vi "Process Data.vi"(7 "Buffer Length":i32, 8 "error in (no error)":errorcluster, 9 "Data":dbl[](array[numeric])=[nan, nan], 10 "XY Plot":refnum<vi>, 11 "Data Rate":i32 caption="ms") -> (0 "error out":errorcluster)   [LabVIEW 2025, in "H1 Plotter.lvlib" / "H1 Velocity.lvclass"]
uses:
  H1 Velocity.lvclass
  H1 Velocity.lvclass/H1 Velocity.ctl
  Users/Public/Documents/Sandia National Labs/TSS Plugin/Tests/XY Plotter.lvlibp/XY  Plotter/XY Plotter.lvclass
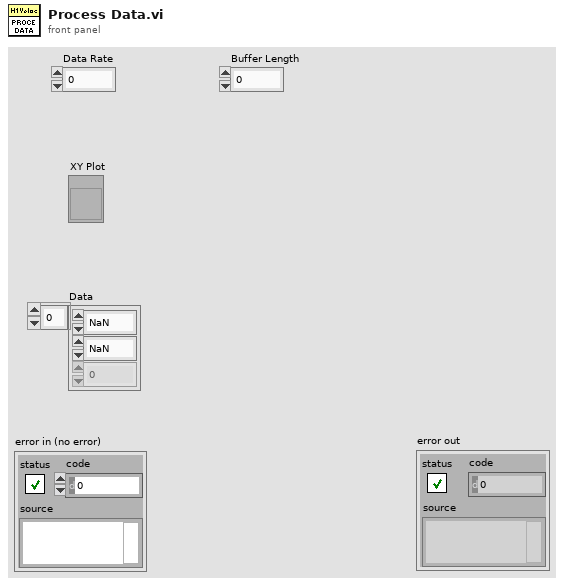
[diagram p1: front panel]
types:
  T1 = cluster{"Active Plot":u32, "XY Data":cluster{"X":dbl[], "Y":dbl[]}}
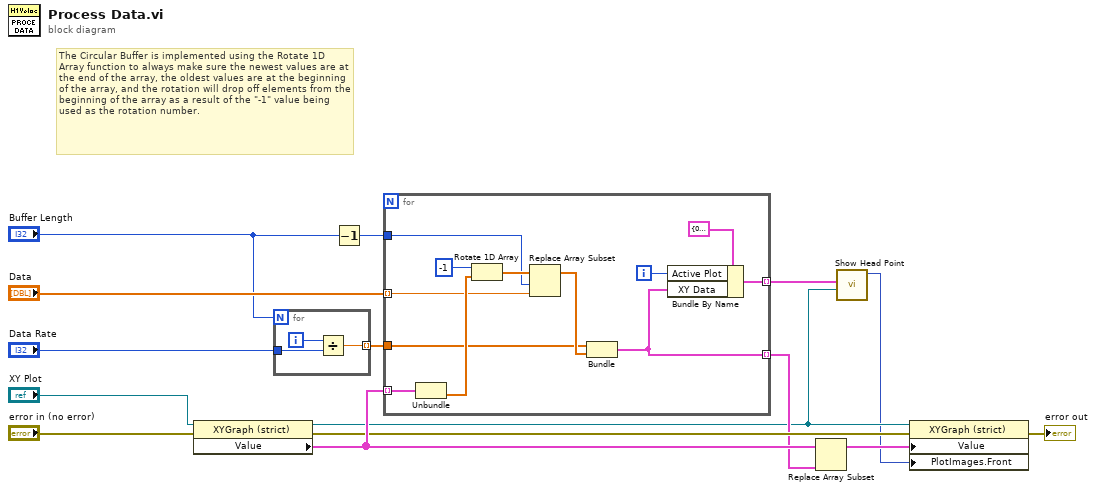
[diagram p0: block diagram]
diagram:
  # "The Circular Buffer is implemented using the Rotate 1D Array function to always make sure the newest values are at the end of the array, the oldest values are at the beginning of the array, and the rotation will drop off elements from the beginning of the array as a result of the \"-1\" value being used as the rotation number."
  n1 = property class="XYGraph (strict)"(reference="XY Plot", error in="error in (no error)") -> (reference out=w8:refnum<vi>, error out=w10:errorcluster, "Value"=w15:cluster{dbl[], dbl[]}[])
  n2 = for {
    N: "Buffer Length" -> [_]
    tunnel: "Data Rate" -> [w17]
    tunnel: [w16] -> w4 mode=indexing
    i -> [w18]
    n3 = Divide(x=w18, y=w17) -> (x/y=w16:dbl)
  }
  n4 = Decrement(x="Buffer Length") -> (x-1=w5:i32)
  n5 = for {
    tunnel: w15 -> [w30] mode=indexing
    tunnel: "Data" -> [w25] mode=indexing
    tunnel: [w21] -> w9 mode=indexing
    tunnel: w5 -> [w26]
    tunnel: [w20] -> w7 mode=indexing
    tunnel: w4 -> [w19]
    i -> [w22]
    n6 = Unbundle(w30) -> (w28:dbl[])  [unwired: 1 out]
    n7 = Rotate 1D Array(1:w28, 2:-1 ("n")) -> (0:w27:dbl[])
    n8 = Replace Array Subset(array=w27, new element=w25, index=w26) -> (w24:dbl[])
    n9 = Bundle(w19, w24) -> (w21:cluster{dbl[], dbl[]})  [unwired: 1 in]
    n10 = Bundle By Name(cluster=T1 {"Active Plot"=0, "XY Data"={"X"=[], "Y"=[]}} ("Dataset"), "Active Plot"=w22, "XY Data"=w21) -> (w20:T1)
  }
  n11 = Replace Array Subset(array=w15, new element=w9) -> (w11:cluster{dbl[], dbl[]}[])  [unwired: 1 in]
  n12 = call "Show Head Point.vi"("XY Plot"=w8, "DataSet"=w7) -> ("picture out"=w6:picture)  [unwired: 7 in, 2 out]
  n13 = property class="XYGraph (strict)"(reference=w8, error in=w10, "Value"=w11, "PlotImages.Front"=w6) -> (error out=→"error out":errorcluster)  [unwired: 1 out]
